vi "Write signal type.vi"(8 "error in (no error)":errorcluster, 10 "signal type":string(combo)="Omit", 11 "DAQNavi_AI in":refnum<class "DAQNavi_AI.lvclass">) -> (0 "error out":errorcluster, 3 "DAQNavi_AI out":refnum<class "DAQNavi_AI.lvclass">)   [LabVIEW 2021, in "DAQNavi_AI.lvclass"]
uses:
  DAQNavi_AI.lvclass
  DAQNavi_AI.lvclass/DAQNavi_AI.ctl
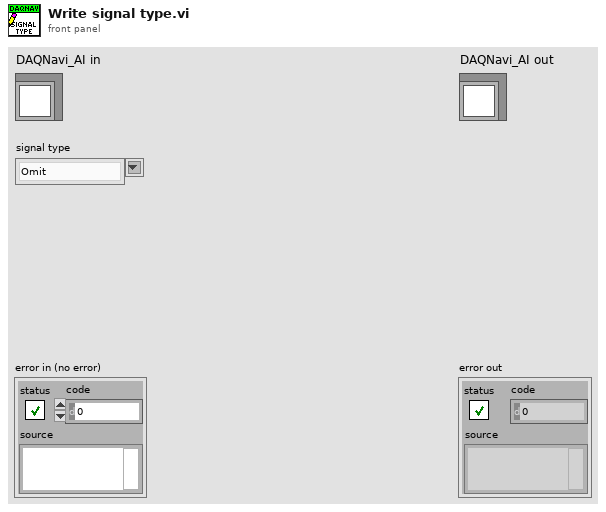
[diagram p1: front panel]
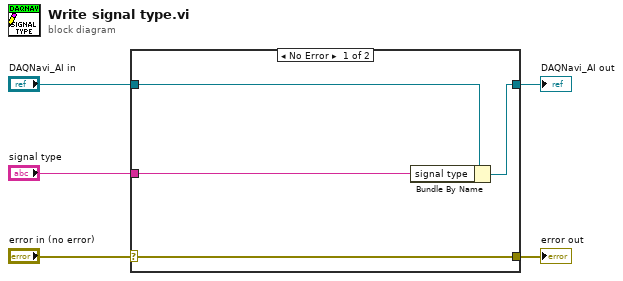
[diagram p0: block diagram]
diagram:
  n1 = case shown="No Error" "error in (no error)" {
    selector: "error in (no error)" -> [w9 w10]
    tunnel: [w9 w10] -> w4
    tunnel: [w7 w11] -> w2
    tunnel: "DAQNavi_AI in" -> [w8 w11]
    tunnel: "signal type" -> [w6 _]
    frame No Error {
      n2 = Bundle By Name(cluster=w8, "signal type"=w6) -> (w7:refnum<class "DAQNavi_AI.lvclass">)
    }
    frame Error {
    }
  }
  "error out" <- w4
  "DAQNavi_AI out" <- w2
